vi "test_header_map.vi"() -> ()   [LabVIEW 2020, in "reqwest_tests.lvlib"]
uses:
  reqwest_tests.lvlib
  Headers/Headers.lvclass
  <vilib>/addons/_JKI Toolkits/Caraya/classes/Assert/Assert.lvclass
  <vilib>/addons/_JKI Toolkits/Caraya/classes/Test/Test.lvclass
panel:
  out "success":bool
  in  "error in (no error)":errorcluster
  out "error out":errorcluster
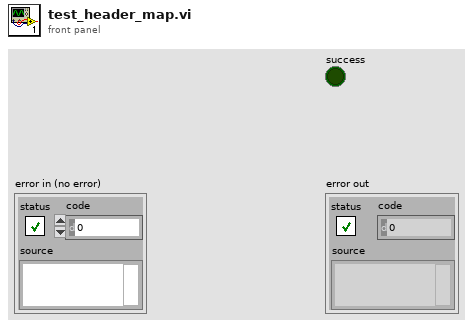
[diagram p1: front panel]
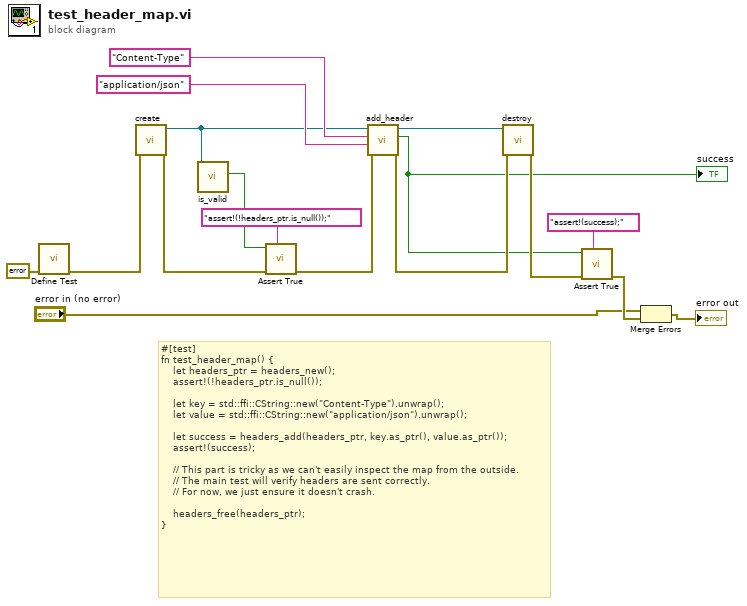
[diagram p0: block diagram]
diagram:
  # "#[test]\nfn test_header_map() {\n    let headers_ptr = headers_new();\n    assert!(!headers_ptr.is_null());\n\n    let key = std::ffi::CString::new(\"Content-Type\").unwrap();\n    let value = std::ffi::CString::new(\"application/json\").unwrap();\n\n    let success = headers_add(headers_ptr, key.as_ptr(), value.as_ptr());\n    assert!(success);\n\n    // This part is tricky as we can't easily inspect the map from the outside.\n    // The main test will verify headers are sent correctly.\n    // For now, we just ensure it doesn't crash.\n\n    headers_free(headers_ptr);\n}"
  n1 = call <vilib>:"Define Test.vi"("error in (no error)"=errorcluster {"status"=FALSE, "code"=0, "source"=""}) -> ("error out"=w10:errorcluster)  [unwired: 9 in, 1 out]
  n2 = call "create.vi"("error in (no error)"=w10) -> ("error out"=w5:errorcluster, "Headers out"=w8:refnum<class "Headers.lvclass">)  [unwired: 9 in]
  n3 = call "is_valid.vi"("Headers in"=w8) -> ("valid-ref?"=w6:bool)  [unwired: 10 in]
  n4 = call <vilib>:"Assert True.vi"("Label"="assert!(!headers_ptr.is_null());", "error in (no error)"=w5, "True?"=w6) -> ("error out"=w4:errorcluster)  [unwired: 7 in, 1 out]
  n5 = call "add_header.vi"("error in (no error)"=w4, "value"="application/json", "key"="Content-Type", "Headers in"=w8) -> ("error out"=w3:errorcluster, "success"=w1:bool, "Headers out"=w2:refnum<class "Headers.lvclass">)  [unwired: 5 in]
  "success" <- w1
  n6 = call "destroy.vi"("error in (no error)"=w3, "Headers in"=w2) -> ("error out"=w17:errorcluster)  [unwired: 9 in]
  n7 = call <vilib>:"Assert True.vi"("Label"="assert!(success);", "error in (no error)"=w17, "True?"=w1) -> ("error out"=w16:errorcluster)  [unwired: 7 in, 1 out]
  n8 = Merge Errors("error in (no error)", w16) -> (→"error out":errorcluster)
